vi "DF003 - CFile Builder Strings.vi"(9 "Language Prefix":string, 10 "Value Row Index":i32, 11 "Input Table (String Array)":string[][](array[string])) -> (3 "Generated Constant Strings":string[](array[string]))   [LabVIEW 2015]
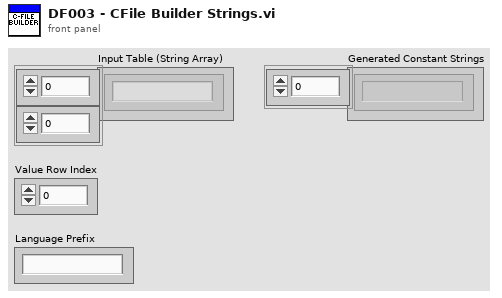
[diagram p1: front panel]
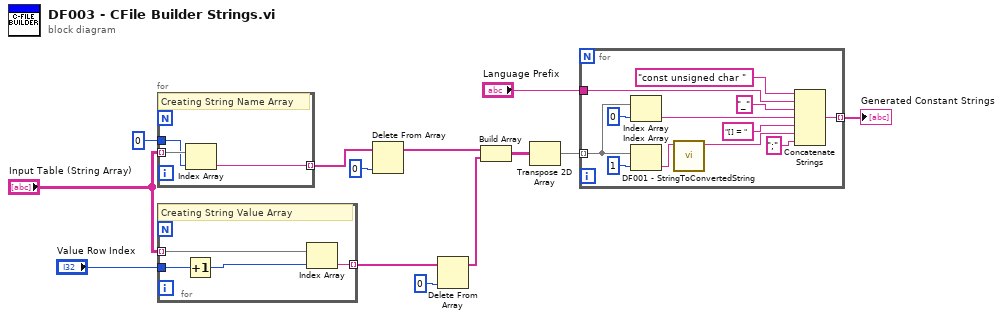
[diagram p0: block diagram]
diagram:
  n1 = for {
    tunnel: "Input Table (String Array)" -> [w16] mode=indexing
    tunnel: [w15] -> w2 mode=indexing
    tunnel: 0 -> [w14]
    # "Creating String Name Array"
    n2 = Index Array(array=w16, index=w14) -> (element=w15:string)
  }
  n3 = for {
    tunnel: "Input Table (String Array)" -> [w20] mode=indexing
    tunnel: [w19] -> w5 mode=indexing
    tunnel: "Value Row Index" -> [w18]
    # "Creating String Value Array"
    n4 = Increment(x=w18) -> (x+1=w17:i32)
    n5 = Index Array(array=w20, index=w17) -> (element=w19:string)
  }
  n6 = Delete From Array(array=w2, index=0) -> (array with subset deleted=w6:string[])  [unwired: 1 in, 1 out]
  n7 = Delete From Array(array=w5, index=0) -> (array with subset deleted=w7:string[])  [unwired: 1 in, 1 out]
  n8 = Build Array(w6, w7) -> (w8:string[][])
  n9 = Transpose 2D Array(2D array=w8) -> (transposed array=w9:string[][])
  n10 = for {
    tunnel: w9 -> [w31] mode=indexing
    tunnel: [w24] -> w12 mode=indexing
    tunnel: "Language Prefix" -> [w22]
    n11 = Index Array(array=w31, index=0) -> (element=w26:string)
    n12 = Index Array(array=w31, index=1) -> (element=w25:string)
    n13 = call "DF001 - StringToConvertedString.vi"("String (Input)"=w25) -> ("Converted String (Output)"=w28:string)  [unwired: 10 in]
    n14 = Concatenate Strings("const unsigned char ", w22, "_" ("string"), w26, "[] = ", w28, ";" ("string")) -> (w24:string)
  }
  "Generated Constant Strings" <- w12
